vi "seqDatareader.vi"(8 "エラー入力":errorcluster) -> (0 "error out":errorcluster, 1 "Seq":string[](array[string]), 2 "Seq_name":string[](array[string]), 3 "output cluster":cluster{string[], string[]}, 5 "Array 3":cluster{string, bool}[](array[cluster]))   [LabVIEW 2018]
panel:
  out "array w/ subset deleted":string[][](array[string])
  out "path":path
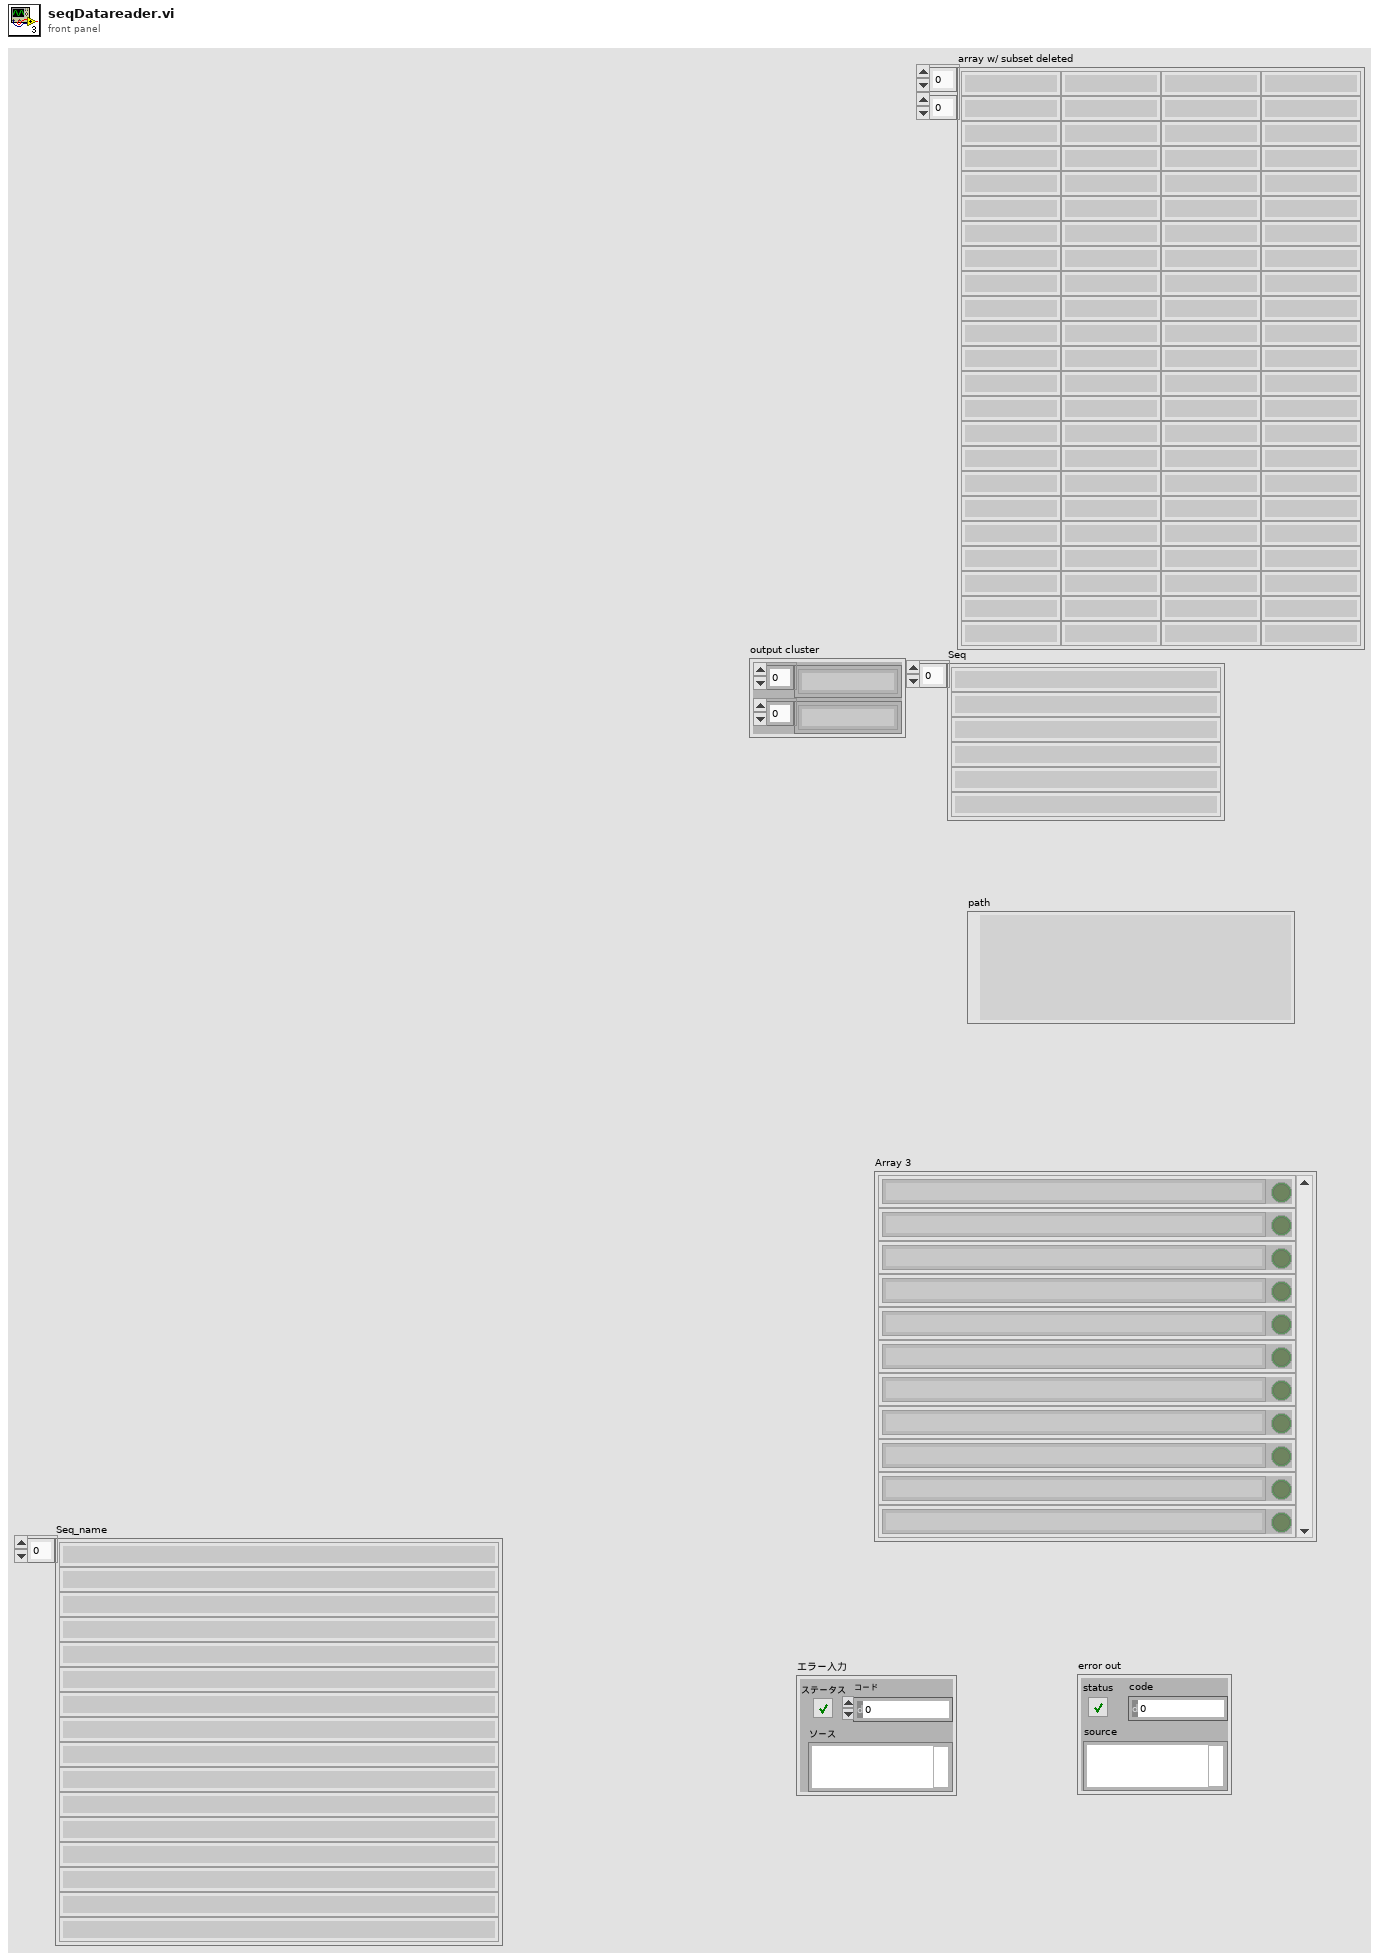
[diagram p1: front panel]
types:
  T1 = enum16{"open", "replace", "create", "open or create", "replace or create", "replace or create with confirmation"}
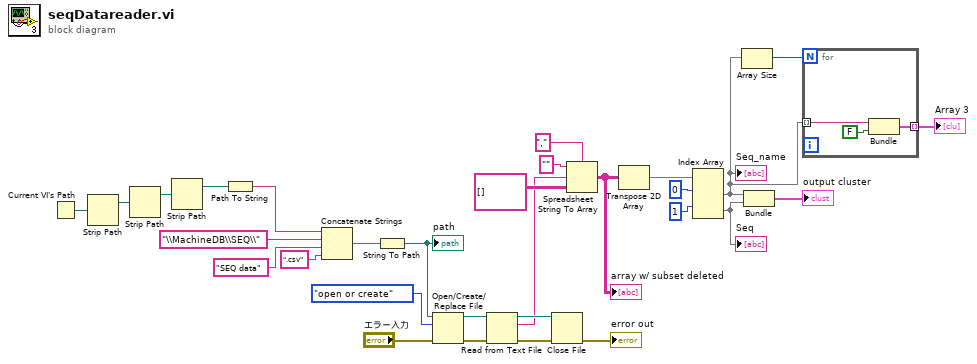
[diagram p0: block diagram]
diagram:
  n1 = Current VI's Path() -> (path=w14:path)
  n2 = Strip Path(path=w14) -> (stripped path=w13:path)  [unwired: 1 out]
  n3 = Strip Path(path=w13) -> (stripped path=w12:path)  [unwired: 1 out]
  n4 = Strip Path(path=w12) -> (stripped path=w11:path)  [unwired: 1 out]
  n5 = Path To String(path=w11) -> (string=w20:string)
  n6 = Concatenate Strings(w20, "\\MachineDB\\SEQ\\" ("string"), "SEQ data" ("string"), ".csv" ("文字列")) -> (w17:string)
  n7 = String To Path(string=w17) -> (path=w25:path)
  "path" <- w25
  n8 = Open/Create/Replace File(file path (use dialog)=w25, error in="エラー入力", operation (0:open)=T1."open or create" ("操作（0:open）")) -> (refnum out=w29:refnum<file>, error out=w30:errorcluster)  [unwired: 3 in, 1 out]
  n9 = Read from Text File(file (use dialog)=w29, error in=w30) -> (refnum out=w26:refnum<file>, text=w22:string, error out=w27:errorcluster)  [unwired: 2 in, 1 out]
  n10 = Close File(refnum=w26, error in=w27) -> (error out=→"error out":errorcluster)  [unwired: 1 out]
  n11 = Spreadsheet String To Array(delimiter (Tab)="," ("デリミタ（タブ）"), format string="" ("形式文字列"), spreadsheet string=w22, array type (2D Dbl)=string[][] [] ("付加配列")) -> (array=w9:string[][])
  "array w/ subset deleted" <- w9
  n12 = Transpose 2D Array(2D array=w9) -> (transposed array=w7:string[][])
  n13 = Index Array(array=w7, index (row) #1=0 ("index (row)"), index (row) #2=1 ("index (row)")) -> (element #1=w1:string[], element #2=w2:string[])  [unwired: 2 in]
  "Seq_name" <- w1
  "Seq" <- w2
  n14 = Array Size(array=w1) -> (size(s)=w4:i32)
  n15 = Bundle(w1, w2) -> (→"output cluster":cluster{string[], string[]})  [unwired: 1 in]
  n16 = for {
    N: w4 -> [_]
    tunnel: w1 -> [w32] mode=indexing
    tunnel: [w33] -> w3 mode=indexing
    n17 = Bundle("Sample ID"=w32, FALSE) -> (w33:cluster{"Sample ID":string, bool})  [unwired: 1 in]
  }
  "Array 3" <- w3
